vi "test http get rejected.vi"(8 "error in (no error)":errorcluster) -> (0 "error out":errorcluster, 3 "body":string)   [LabVIEW 2020, in "MCP Server tests.lvlib"]
doc: "A GET on the MCP endpoint must be answered with 405 Method Not Allowed, an Allow: POST header and a JSON-RPC error with code -32600."
uses:
  MCP Server tests.lvlib
  <vilib>/addons/_JKI Toolkits/Caraya/classes/Test/Test.lvclass
  <vilib>/addons/_JKI Toolkits/Caraya/classes/Assert/Assert.lvclass
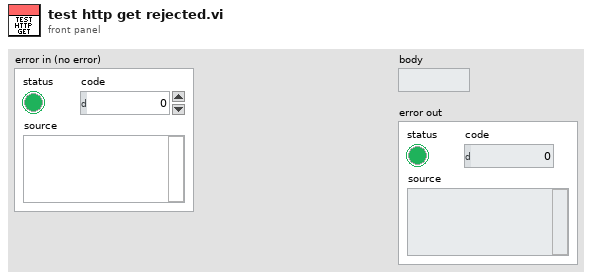
[diagram p1: front panel]
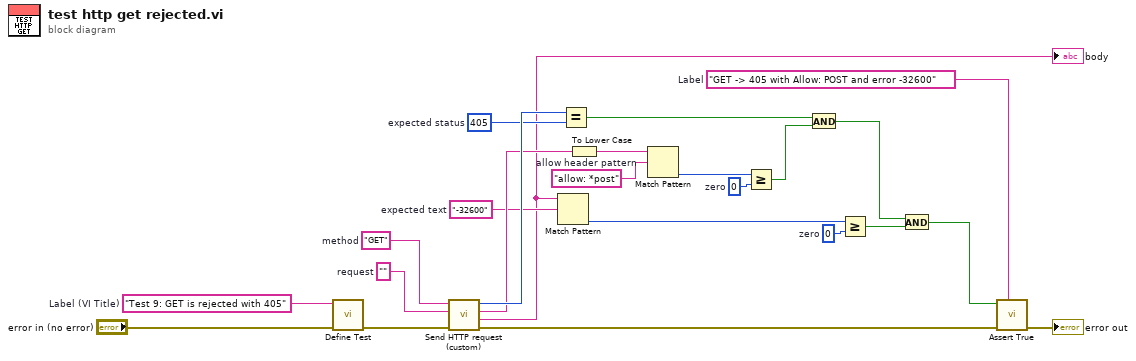
[diagram p0: block diagram]
diagram:
  w3 = "GET -> 405 with Allow: POST and error -32600"  # Label
  w10 = 0  # zero
  w12 = "-32600"  # expected text
  w13 = 0  # zero
  w15 = "allow: *post"  # allow header pattern
  w18 = 405  # expected status
  w21 = ""  # request
  w22 = "GET"  # method
  w24 = "Test 9: GET is rejected with 405"  # Label (VI Title)
  n1 = call <vilib>:"Define Test.vi"("error in (no error)"="error in (no error)", "Label (VI Title)"=w24) -> ("error out"=w20:errorcluster)  [unwired: 8 in, 1 out]
  n2 = call "Send HTTP request (custom).vi"("error in (no error)"=w20, "request"=w21, "method"=w22) -> ("error out"=w4:errorcluster, "response"=w2:string, "headers"=w17:string, "status code"=w19:i32)  [unwired: 5 in]
  "body" <- w2
  n3 = Match Pattern(string=w2, regular expression=w12) -> (offset past match=w11:i32)  [unwired: 1 in, 3 out]
  n4 = Equal?(x=w19, y=w18) -> (x = y?=w9:bool)
  n5 = To Lower Case(string=w17) -> (all lower case string=w16:string)
  n6 = Match Pattern(string=w16, regular expression=w15) -> (offset past match=w14:i32)  [unwired: 1 in, 3 out]
  n7 = Greater Or Equal?(x=w14, y=w13) -> (x >= y?=w8:bool)
  n8 = And(x=w9, y=w8) -> (x .and. y?=w7:bool)
  n9 = Greater Or Equal?(x=w11, y=w10) -> (x >= y?=w6:bool)
  n10 = And(x=w7, y=w6) -> (x .and. y?=w5:bool)
  n11 = call <vilib>:"Assert True.vi"("Label"=w3, "error in (no error)"=w4, "True?"=w5) -> ("error out"=→"error out":errorcluster)  [unwired: 7 in, 1 out]
